vi "Defaults.vi"() -> (2 "Defaults":T1)   [LabVIEW 2020, in "VolatusGUIElements.lvlib" / "DigitalButtonControl.lvclass"]
uses:
  DigitalButtonControl.lvclass
  JSON.ctl
  DigitalButtonControl.lvclass/DigitalButtonControl.ctl
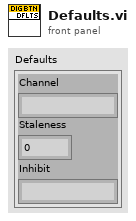
[diagram p1: front panel]
types:
  T1 = typedef "VolatusGUIElements.lvlib/DigitalButtonControl.lvclass/JSON.ctl" = cluster{"Channel":string, "Staleness":dbl, "Inhibit":string}
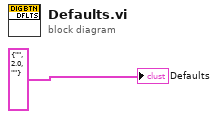
[diagram p0: block diagram]
diagram:
  "Defaults" <- T1 {"Channel"="", "Staleness"=2.0, "Inhibit"=""} ("JSON")
